vi "pinMode.Soft_Tone.vi"(8 "error in (no error)":errorcluster, 11 "RPi Pin":T1=enum."GPIO2_I2C1_SDA_Pin3") -> (0 "error out":errorcluster, 3 "RPi Pin out":T1=enum."GPIO2_I2C1_SDA_Pin3")   [LabVIEW 2020, in "wiringPi.lvlib"]
doc: "<b>_______________________________________________________________</b>\n** Author: Juan José Villacorta\n** LabVIEW wrapper for C library <b> wiringPi </b>,\n** https://github.com/WiringPi/WiringPi\n<b>_______________________________________________________________</b>\n\n\n/*\n * pinMode:\n * Sets the mode of a pin to be input, output or PWM output\n *********************************************************************************\n// Pin modes\n#define INPUT 0\n#define OUTPUT 1\n#define PWM_OUTPUT 2\n#define PWM_MS_OUTPUT 8\n#define PWM_BAL_OUTPUT 9\n#define GPIO_CLOCK 3\n#define SOFT_PWM_OUTPUT 4\n#define SOFT_TONE_OUTPUT 5\n#define PWM_TONE_OUTPUT 6\n#define PM_OFF 7 // to input / release line"
uses:
  wiringPi.lvlib
  Type Defs/GPIO Mode.ctl
  Type Defs/GPIO Pins.ctl
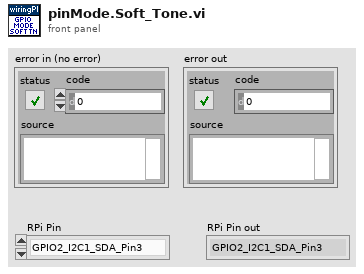
[diagram p1: front panel]
types:
  T1 = typedef "wiringPi.lvlib/GPIO Pins.ctl" = enum32{"GPIO0_I2C0_SDA_Pin27", "GPIO1_I2C0_SDA1_Pin28", "GPIO2_I2C1_SDA_Pin3", "GPIO3_I2C1_SCL_Pin5", "GPIO4_GPCLK0_Pin7", "GPIO5_GPCLK1_Pin29", "GPIO6_GPCLK2_Pin31", "GPIO7_SPI_CE1_N_Pin26", "GPIO8_SPI_CE0_N_Pin24", "GPIO9_SPI0_MISO_Pin21", "GPIO10_SPI0_MOSI_Pin19", "GPIO11_SPI0_CLK_Pin23", "GPIO12_PWM0_Pin32", "GPIO13_PWM1_Pin33", "GPIO14_TXD0_Pin8", "GPIO15_RXD0_Pin10", "GPIO16_Pin36", "GPIO17_Pin11", "GPIO18_PWM0_Pin12", "GPIO19_PWM1_Pin35", "GPIO20_GPCLK0_Pin38", "GPIO21_GPCLK1_Pin40", "GPIO22_Pin15", "GPIO23_Pin16", "GPIO24_Pin18", "GPIO25_Pin22", "GPIO26_Pin37", "GPIO27_Pin13"}
  T2 = typedef "wiringPi.lvlib/GPIO Mode.ctl" = u16
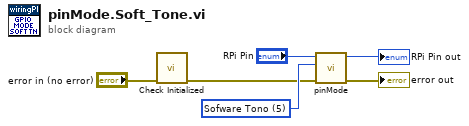
[diagram p0: block diagram]
diagram:
  w3 = T2 5 items=["Input"=0, "Output"=1, "PWM"=2, "PWM Mark/Space"=8, "PWM Balanced"=9, "Clock"=3, "Software PWM"=4, "Sofware Tono"=5, "PWM Tone"=6, "Off"=7] ("Mode")
  n1 = call "Check Initialized.vi"("error in (no error)"="error in (no error)") -> ("error out"=w1:errorcluster)  [unwired: 10 in]
  n2 = call "pinMode.vi"("error in (no error)"=w1, "Mode"=w3, "RPi Pin"="RPi Pin") -> ("error out"=→"error out":errorcluster, "RPi Pin out"=→"RPi Pin out":T1)  [unwired: 7 in]
